vi "Test Find Account.vi"() -> ()   [LabVIEW 2026]
doc: "Caraya unit test for Find Account.vi, generated by lvai_generate_test.\n\nOne static subVI call per case. Every assertion takes its error in from Define Test rather than from the assertion before it, so a failing case cannot stop a later one - chaining them silently loses cases, measured.\n\nThe error cluster carries the FIRST failure only. Read the JUnit report for all of them."
uses:
  <vilib>/addons/_JKI Toolkits/Caraya/classes/Test/Test.lvclass
  <vilib>/addons/_JKI Toolkits/Caraya/classes/Assert/Assert.lvclass
panel:
  out "error out":errorcluster
  in  "error in":errorcluster
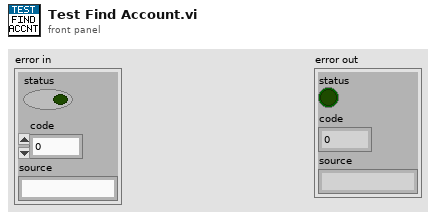
[diagram p1: front panel]
types:
  T1 = cluster{"Account Number":string, "First Name":string, "Last Name":string, "Balance":dbl}
  T2 = cluster{"Account Number":string, "First Name":string, "Last Name":string, "Balance":dbl}[]
  T3 = typedef "ATM Account.ctl" = cluster{"Account Number":string, "First Name":string, "Last Name":string, "Balance":dbl}
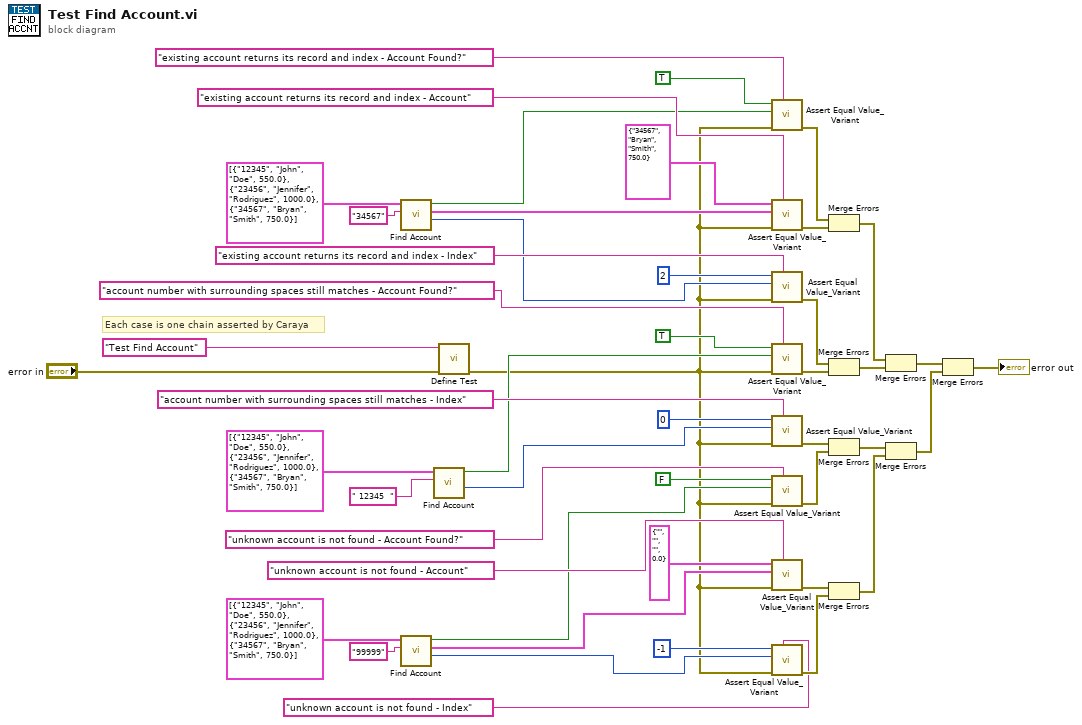
[diagram p0: block diagram]
diagram:
  # "Each case is one chain asserted by Caraya"
  n1 = call "Find Account.vi"("Account Number"="34567", "Accounts"=T2 [{"Account Number"="12345", "First Name"="John", "Last Name"="Doe", "Balance"=550.0}, {"Account Number"="23456", "First Name"="Jennifer", "Last Name"="Rodriguez", "Balance"=1000.0}, {"Account Number"="34567", "First Name"="Bryan", "Last Name"="Smith", "Balance"=750.0}]) -> ("Index"=w8:i32, "Account"=w7:T3, "Account Found?"=w6:bool)  [unwired: 6 in, 1 out]
  n2 = call "Find Account.vi"("Account Number"="99999", "Accounts"=T2 [{"Account Number"="12345", "First Name"="John", "Last Name"="Doe", "Balance"=550.0}, {"Account Number"="23456", "First Name"="Jennifer", "Last Name"="Rodriguez", "Balance"=1000.0}, {"Account Number"="34567", "First Name"="Bryan", "Last Name"="Smith", "Balance"=750.0}]) -> ("Index"=w32:i32, "Account"=w31:T3, "Account Found?"=w30:bool)  [unwired: 6 in, 1 out]
  n3 = call "Find Account.vi"("Account Number"=" 12345  ", "Accounts"=T2 [{"Account Number"="12345", "First Name"="John", "Last Name"="Doe", "Balance"=550.0}, {"Account Number"="23456", "First Name"="Jennifer", "Last Name"="Rodriguez", "Balance"=1000.0}, {"Account Number"="34567", "First Name"="Bryan", "Last Name"="Smith", "Balance"=750.0}]) -> ("Index"=w21:i32, "Account Found?"=w20:bool)  [unwired: 6 in, 2 out]
  n4 = call <vilib>:"Define Test.vi"("error in (no error)"="error in", "Label (VI Title)"="Test Find Account") -> ("error out"=w3:errorcluster)  [unwired: 8 in, 1 out]
  n5 = call <vilib>:"Assert Equal Value_Variant.vi"("Label"="existing account returns its record and index - Account Found?", "error in (no error)"=w3, "Actual"=w6, "Expected"=TRUE ("expected 1")) -> ("error out"=w11:errorcluster)  [unwired: 6 in, 1 out]
  n6 = call <vilib>:"Assert Equal Value_Variant.vi"("Label"="existing account returns its record and index - Account", "error in (no error)"=w3, "Actual"=w7, "Expected"=T1 {"Account Number"="34567", "First Name"="Bryan", "Last Name"="Smith", "Balance"=750.0} ("expected 2")) -> ("error out"=w14:errorcluster)  [unwired: 6 in, 1 out]
  n7 = call <vilib>:"Assert Equal Value_Variant.vi"("Label"="existing account returns its record and index - Index", "error in (no error)"=w3, "Actual"=w8, "Expected"=2 ("expected 3")) -> ("error out"=w17:errorcluster)  [unwired: 6 in, 1 out]
  n8 = call <vilib>:"Assert Equal Value_Variant.vi"("Label"="account number with surrounding spaces still matches - Account Found?", "error in (no error)"=w3, "Actual"=w20, "Expected"=TRUE ("expected 4")) -> ("error out"=w24:errorcluster)  [unwired: 6 in, 1 out]
  n9 = call <vilib>:"Assert Equal Value_Variant.vi"("Label"="account number with surrounding spaces still matches - Index", "error in (no error)"=w3, "Actual"=w21, "Expected"=0 ("expected 5")) -> ("error out"=w27:errorcluster)  [unwired: 6 in, 1 out]
  n10 = call <vilib>:"Assert Equal Value_Variant.vi"("Label"="unknown account is not found - Account Found?", "error in (no error)"=w3, "Actual"=w30, "Expected"=FALSE ("expected 6")) -> ("error out"=w35:errorcluster)  [unwired: 6 in, 1 out]
  n11 = call <vilib>:"Assert Equal Value_Variant.vi"("Label"="unknown account is not found - Account", "error in (no error)"=w3, "Actual"=w31, "Expected"=T1 {"Account Number"="", "First Name"="", "Last Name"="", "Balance"=0.0} ("expected 7")) -> ("error out"=w38:errorcluster)  [unwired: 6 in, 1 out]
  n12 = call <vilib>:"Assert Equal Value_Variant.vi"("Label"="unknown account is not found - Index", "error in (no error)"=w3, "Actual"=w32, "Expected"=-1 ("expected 8")) -> ("error out"=w41:errorcluster)  [unwired: 6 in, 1 out]
  n13 = Merge Errors(w11, w14) -> (w42:errorcluster)
  n14 = Merge Errors(w17, w24) -> (w43:errorcluster)
  n15 = Merge Errors(w27, w35) -> (w44:errorcluster)
  n16 = Merge Errors(w38, w41) -> (w45:errorcluster)
  n17 = Merge Errors(w42, w43) -> (w46:errorcluster)
  n18 = Merge Errors(w44, w45) -> (w47:errorcluster)
  n19 = Merge Errors(w46, w47) -> (→"error out":errorcluster)
